vi "Set Labels and Visibility.vi"(1 "error In":errorcluster, 2 "Offset Refnum":refnum<vi>, 3 "Type":T1, 4 "Amplitude Refnum":refnum<vi>, 5 "Periods Renum":refnum<vi>, 6 "Phase Refnum":refnum<vi>, 7 "Function Refnum":refnum<vi>) -> (0 "error out":errorcluster)   [LabVIEW 2012, in "Waveform Control.xctl"]
doc: "Set the captions and visibility of the function generator controls depending on the selected function"
uses:
  Waveform Control.xctl
  Function Types.ctl
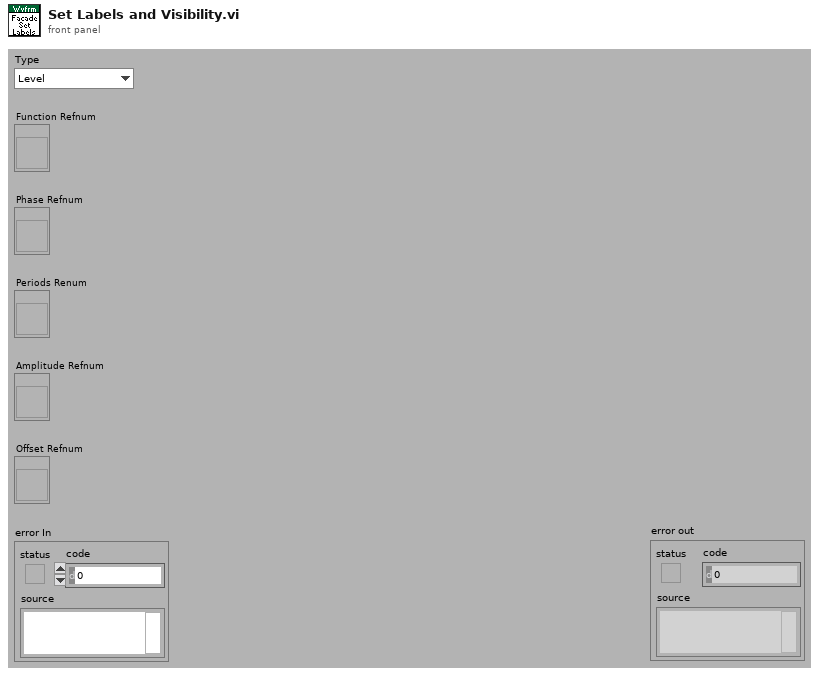
[diagram p1: front panel]
types:
  T1 = typedef "Waveform Control.xctl/Function Types.ctl" = enum16{"Level", "Sine", "Triangle", "Ramp", "Saw Tooth", "Square", "Function"}
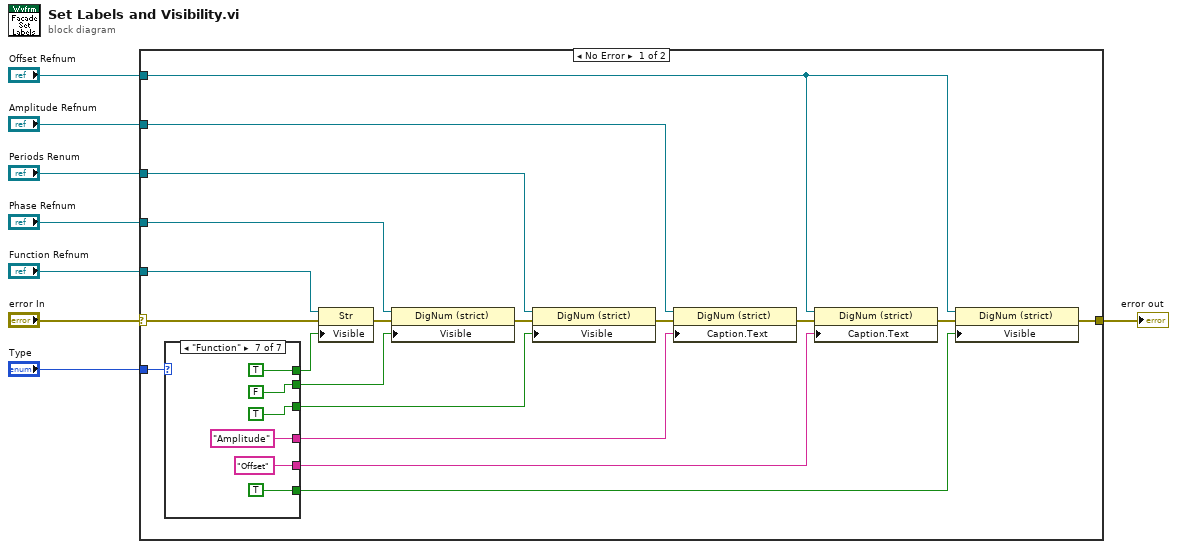
[diagram p0: block diagram]
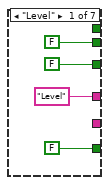
[diagram p2: hidden frame]
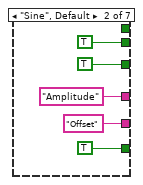
[diagram p3: hidden frame]
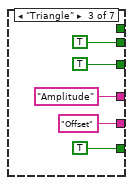
[diagram p4: hidden frame]
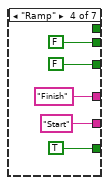
[diagram p5: hidden frame]
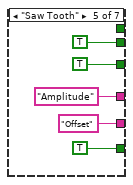
[diagram p6: hidden frame]
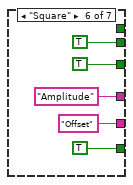
[diagram p7: hidden frame]
diagram:
  n1 = case shown="No Error" "error In" {
    selector: "error In" -> [w21 w63]
    tunnel: "Type" -> [w15 _]
    tunnel: "Function Refnum" -> [w14 _]
    tunnel: "Phase Refnum" -> [w13 _]
    tunnel: "Periods Renum" -> [w12 _]
    tunnel: "Amplitude Refnum" -> [w11 _]
    tunnel: "Offset Refnum" -> [w10 _]
    tunnel: [w9 w63] -> w1
    frame No Error {
      n2 = case shown="\"Function\"" w15 {
        tunnel: [_ _ _ _ _ _ TRUE] -> w16
        tunnel: [FALSE TRUE TRUE FALSE TRUE TRUE FALSE] -> w17
        tunnel: [FALSE TRUE TRUE FALSE TRUE TRUE TRUE] -> w18
        tunnel: ["Level" "Amplitude" "Amplitude" "Finish" "Amplitude" "Amplitude" "Amplitude"] -> w19
        tunnel: [_ "Offset" "Offset" "Start" "Offset" "Offset" "Offset"] -> w20
        tunnel: [FALSE TRUE TRUE TRUE TRUE TRUE TRUE] -> w27
        frame "Level" {
        }
        frame "Sine", Default {
        }
        frame "Triangle" {
        }
        frame "Ramp" {
        }
        frame "Saw Tooth" {
        }
        frame "Square" {
        }
        frame "Function" {
        }
      }
      n3 = property on="Property Node" class="Str"(reference=w14, error in=w21, "Visible"=w16) -> (error out=w22:errorcluster)  [unwired: 1 out]
      n4 = property on="Property Node" class="DigNum (strict)"(reference=w13, error in=w22, "Visible"=w17) -> (error out=w23:errorcluster)  [unwired: 1 out]
      n5 = property on="Property Node" class="DigNum (strict)"(reference=w12, error in=w23, "Visible"=w18) -> (error out=w24:errorcluster)  [unwired: 1 out]
      n6 = property on="Property Node" class="DigNum (strict)"(reference=w11, error in=w24, "Caption.Text"=w19) -> (error out=w25:errorcluster)  [unwired: 1 out]
      n7 = property on="Property Node" class="DigNum (strict)"(reference=w10, error in=w25, "Caption.Text"=w20) -> (error out=w26:errorcluster)  [unwired: 1 out]
      n8 = property on="Property Node" class="DigNum (strict)"(reference=w10, error in=w26, "Visible"=w27) -> (error out=w9:errorcluster)  [unwired: 1 out]
    }
    frame Error {
    }
  }
  "error out" <- w1
